vi "2636 EPSC fully synced version.vi"() -> ()   [LabVIEW 2023]
uses:
  <instrlib>/Keithley 2600 Series/Public/Channel.ctl
  <instrlib>/Keithley 2600 Series/Keithley 2600 Series.lvlib
  <userlib>/_OpenG.lib/time/time.llb/openg_time.lvlib
panel:
  in  "error in (no error)":errorcluster
  in  "Log Time After Pulses (s)":dbl=0.5 format="%#_13g"
  in  "Log Time Before Pulses (s)":dbl=0.5 format="%#_13g"
  in  "Auto Enable Output":bool=TRUE
  in  "Reset":bool=TRUE
  in  "Error Query":bool
  out "Pulsed IV Filename Out":path caption="Filename Out"
  in  "Pulsed IV Filename":path=path "C:/Data/pulse_I_V.lvm" caption="Filename"
  out "Pulse IV":cluster{"X":dbl[], "Y":dbl[]}[](graph)
  out "I_ds Log Filename Out":path caption="Filename Out"
  in  "I_ds Log Filename":path=path "C:/Data/I_ds_vs_time.lvm" caption="Filename"
  out "Data":dbl[](array[numeric])
  out "Result Chart":dynamicdata(graph)
  out "error out":errorcluster
  out "Complete?":bool
  out "Overflow?":bool
  in  "Stop":bool
  in  "Pulse Duration (s)":dbl=0.01
  in  "Post-Pulse Duration (s)":dbl=0.05
  in  "Pre-Pulse Duration (s)":dbl=0.05
  in  "Buffer size":u32=1024
  in  "Pulse Number":u32=10
  in  "Drain Source Channel":T1=enum."Channel B"
  in  "V_ds(V)":dbl=0.01
  in  "I_ds NPLC":dbl=0.1
  in  "I_ds Range (A)":dbl=1e-06
  in  "I pulse Range (A)":dbl=1e-06
  in  "I pulse NPLC":dbl=0.1
  in  "Pulse Level (V)":dbl=15.0
  in  "Pulse Channel":T1
  in  "2636 Address":refnum<visa-resource-name>="GPIB0::26::INSTR"
  # "Synaptic EPSC Measurement (Three-terminal Devices)"
  # "by JHC (20250322)"
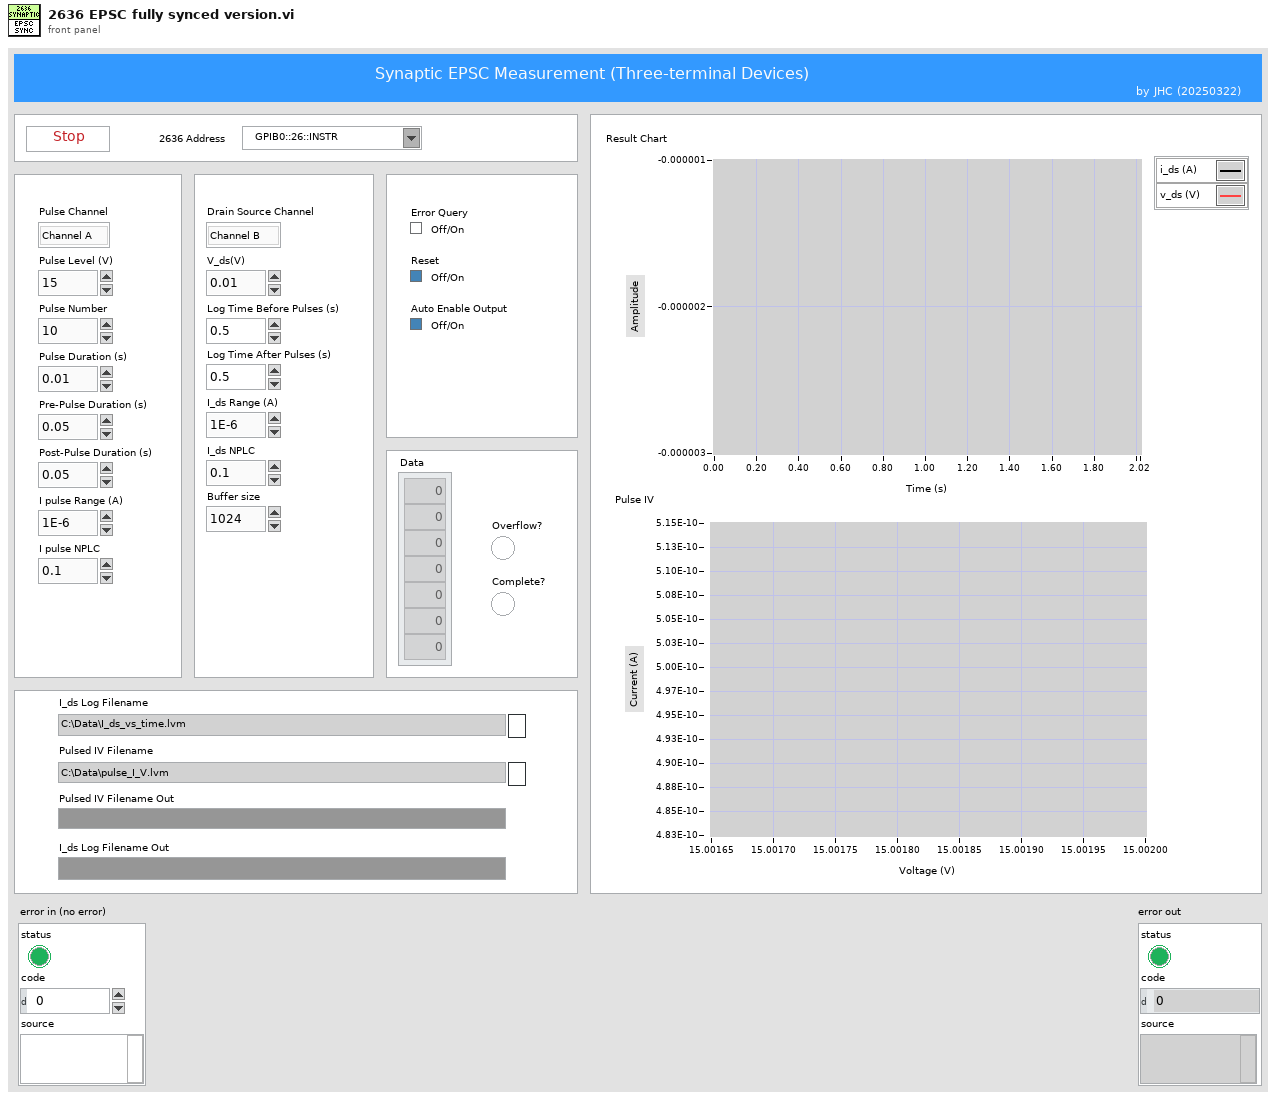
[diagram p1: front panel]
types:
  T1 = typedef "Keithley 2600 Series.lvlib/Channel.ctl" = enum32{"Channel A", "Channel B"}
  T2 = enum16{"None/Disconnect", "Digital I/O Trigger", "TSP-Link Trigger", "LAN Trigger", "Blender", "Timer Expired", "Front Panel Trigger", "Software Trigger", "SMU Sweeping", "SMU Armed", "SMU Source Complete", "SMU Measure Complete", "SMU Pulse Complete", "SMU Sweep Complete", "SMU Idle"}
  T3 = enum16{"Current", "Voltage", "IV", "Resistance", "Power"}
  T4 = enum32{"ASCII", "Real 32", "Real 64", "Single Precision Real", "Double Precision Real"}
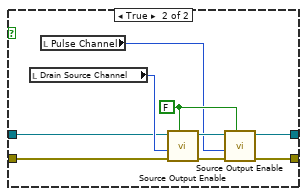
[diagram p2: hidden frame]
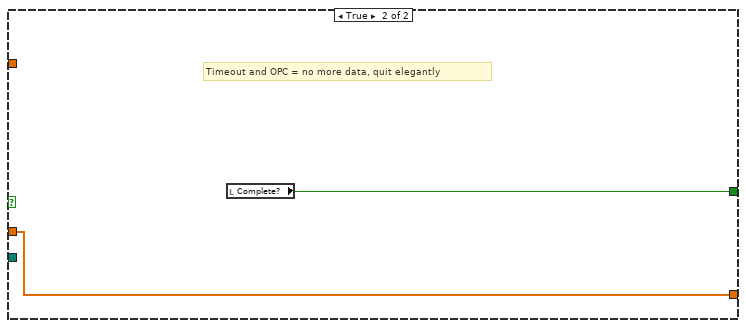
[diagram p5: hidden frame]
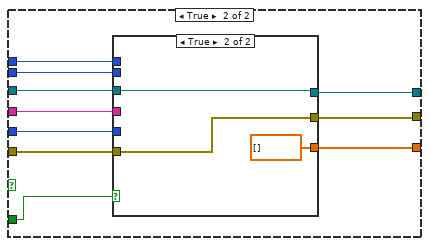
[diagram p8: hidden frame]
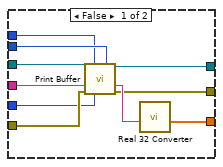
[diagram p9: hidden frame]
diagram:
  w19 = sgl[] [] ("Data Array Out")
  w22 = u16 1 items=["Channel A", "Channel B"] ("Channel (Channel A)")
  w23 = u16 0 items=["Channel A", "Channel B"] ("Channel (Channel A)")
  w39 = u16 0 items=["Current", "Voltage", "Resistance", "Power"] ("Function (Current)")
  w47 = u16 2 items=["Channel A", "Channel B", "Channels A & B", "User"] ("Screen (Channels A & B)")
  # "Wait 1s"
  # "Start Pulse SMU"
  # "Start DS SMU"
  n1 = call <instrlib>:"Initialize.vi"("Reset (True)"="Reset", "error in (no error)"="error in (no error)", "Error Query (False)"="Error Query", "ID Query (True)"=TRUE, "VISA resource name"="2636 Address") -> ("error out"=w2:errorcluster, "VISA resource name out"=w5:refnum<visa-resource-name>)  [unwired: 5 in]
  n2 = call <instrlib>:"Error Queue Clear.vi"("error in (no error)"=w2, "VISA resource name"=w5) -> ("error out"=w3:errorcluster, "VISA resource name out"=w4:refnum<visa-resource-name>)  [unwired: 6 in, 2 out]
  n3 = call <instrlib>:"Abort SMU Op.vi"("error in"=w3, "Channel (Channel A)"=w23, "VISA resource name"=w4) -> ("error out"=w24:errorcluster, "VISA resource name out"=w25:refnum<visa-resource-name>)  [unwired: 5 in, 2 out]
  n4 = call <instrlib>:"Abort SMU Op.vi"("error in"=w24, "Channel (Channel A)"=w22, "VISA resource name"=w25) -> ("error out"=w20:errorcluster, "VISA resource name out"=w21:refnum<visa-resource-name>)  [unwired: 5 in, 2 out]
  n5 = call <instrlib>:"Reset SMU.vi"("SMU B (No)"="Reset", "SMU A (No)"="Reset", "error in (no error)"=w20, "VISA resource name"=w21) -> ("error out"=w86:errorcluster, "VISA resource name out"=w87:refnum<visa-resource-name>)  [unwired: 4 in, 2 out]
  n6 = flat-sequence {
    tunnel: w87 -> [w120]
    tunnel: w86 -> [w119]
    tunnel: [w101] -> w85
    tunnel: [w100] -> w84
    tunnel: w85 -> [w143]
    tunnel: w84 -> [w144]
    tunnel: [w142] -> w83
    tunnel: [w141] -> w82
    tunnel: w83 -> [w184]
    tunnel: w82 -> [w182]
    tunnel: [w163] -> w81
    tunnel: [w162] -> w80
    tunnel: w81 -> [w262]
    tunnel: w80 -> [w261]
    tunnel: [w229] -> w79
    tunnel: [w228] -> w78
    tunnel: [w214] -> w77
    tunnel: w79 -> [w295]
    tunnel: w78 -> [w296]
    tunnel: w77 -> [w318]
    tunnel: [w299] -> w76
    tunnel: [w298] -> w75
    tunnel: w76 -> [w326]
    tunnel: w75 -> [w325]
    tunnel: [w322] -> w44
    tunnel: [w321] -> w43
    frame #0 {
      w108 = enum32{"Current", "Voltage"}."Current" ("Function (Current)")
      w109 = FALSE ("Autorange (On)")
      w89 = enum32{"Current", "Voltage"}."Voltage" ("Function (Current)")
      # "Init Pulse Gate Channel"
      n7 = call <instrlib>:"Source Function.vi"("Function (Current)"=w89, "error in (no error)"=w119, "Channel (Channel A)"="Pulse Channel", "VISA resource name"=w120) -> ("error out"=w121:errorcluster, "VISA resource name out"=w122:refnum<visa-resource-name>)  [unwired: 4 in, 2 out]
      n8 = call <instrlib>:"Source Level.vi"("Level (0.000)"=0.0, "Function (Current)"=w89, "error in (no error)"=w121, "Channel (Channel A)"="Pulse Channel", "VISA resource name"=w122) -> ("error out"=w117:errorcluster, "VISA resource name out"=w118:refnum<visa-resource-name>)  [unwired: 3 in, 2 out]
      n9 = call <instrlib>:"Source Autorange.vi"("Autorange (On)"=w109, "Function (Current)"=w89, "error in (no error)"=w117, "Channel (Channel A)"="Pulse Channel", "VISA resource name"=w118) -> ("error out"=w115:errorcluster, "VISA resource name out"=w116:refnum<visa-resource-name>)  [unwired: 3 in, 2 out]
      n10 = local read "Pulse Level (V)"() -> (w88:dbl)
      n11 = call <instrlib>:"Source Autorange.vi"("Autorange (On)"=w109, "Function (Current)"=w108, "error in (no error)"=w115, "Channel (Channel A)"="Pulse Channel", "VISA resource name"=w116) -> ("error out"=w96:errorcluster, "VISA resource name out"=w98:refnum<visa-resource-name>)  [unwired: 3 in, 2 out]
      n12 = call <instrlib>:"Source Range.vi"("Range (1.000)"=w88, "Function (Current)"=w89, "error in (no error)"=w96, "Channel (Channel A)"="Pulse Channel", "VISA resource name"=w98) -> ("error out"=w95:errorcluster, "VISA resource name out"=w97:refnum<visa-resource-name>)  [unwired: 3 in, 2 out]
      n13 = call <instrlib>:"Measure NPLC.vi"("NPLC (1.000)"="I pulse NPLC", "error in (no error)"=w95, "Channel (Channel A)"="Pulse Channel", "VISA resource name"=w97) -> ("error out"=w113:errorcluster, "VISA resource name out"=w110:refnum<visa-resource-name>)  [unwired: 4 in, 2 out]
      n14 = call <instrlib>:"Measure Autorange.vi"("Autorange (On)"=w109, "Function (Current)"=w89, "error in (no error)"=w113, "Channel (Channel A)"="Pulse Channel", "VISA resource name"=w110) -> ("error out"=w112:errorcluster, "VISA resource name out"=w111:refnum<visa-resource-name>)  [unwired: 3 in, 2 out]
      n15 = call <instrlib>:"Measure Autorange.vi"("Autorange (On)"=w109, "Function (Current)"=w108, "error in (no error)"=w112, "Channel (Channel A)"="Pulse Channel", "VISA resource name"=w111) -> ("error out"=w94:errorcluster, "VISA resource name out"=w93:refnum<visa-resource-name>)  [unwired: 3 in, 2 out]
      n16 = call <instrlib>:"Measure Range.vi"("Range (1.000)"=w88, "Function (Current)"=w89, "error in (no error)"=w94, "Channel (Channel A)"="Pulse Channel", "VISA resource name"=w93) -> ("error out"=w91:errorcluster, "VISA resource name out"=w92:refnum<visa-resource-name>)  [unwired: 3 in, 2 out]
      n17 = call <instrlib>:"Measure Range.vi"("Range (1.000)"="I pulse Range (A)", "Function (Current)"=w108, "error in (no error)"=w91, "Channel (Channel A)"="Pulse Channel", "VISA resource name"=w92) -> ("error out"=w106:errorcluster, "VISA resource name out"=w105:refnum<visa-resource-name>)  [unwired: 3 in, 2 out]
      n18 = call <instrlib>:"Measure Sense Mode.vi"("error in (no error)"=w106, "Channel (Channel A)"="Pulse Channel", "VISA resource name"=w105) -> ("error out"=w103:errorcluster, "VISA resource name out"=w104:refnum<visa-resource-name>)  [unwired: 2 in, 5 out]
      n19 = call <instrlib>:"Measure Autozero.vi"("Autozero (Auto)"=enum32{"Off", "Once", "Auto"}."Once", "error in (no error)"=w103, "Channel (Channel A)"="Pulse Channel", "VISA resource name"=w104) -> ("error out"=w100:errorcluster, "VISA resource name out"=w101:refnum<visa-resource-name>)  [unwired: 1 in, 5 out]
    }
    frame #1 {
      w126 = 0.0 ("Interval (0.000)")
      w146 = enum32{"Current", "Voltage"}."Current" ("Function (Current)")
      w145 = FALSE ("Autorange (On)")
      w132 = enum32{"Current", "Voltage"}."Voltage" ("Function (Current)")
      # "Init Drain Source Channel"
      n20 = call <instrlib>:"Source Function.vi"("Function (Current)"=w132, "error in (no error)"=w144, "Channel (Channel A)"="Drain Source Channel", "VISA resource name"=w143) -> ("error out"=w160:errorcluster, "VISA resource name out"=w161:refnum<visa-resource-name>)  [unwired: 4 in, 2 out]
      n21 = call <instrlib>:"Source Level.vi"("Level (0.000)"="V_ds(V)", "Function (Current)"=w132, "error in (no error)"=w160, "Channel (Channel A)"="Drain Source Channel", "VISA resource name"=w161) -> ("error out"=w158:errorcluster, "VISA resource name out"=w159:refnum<visa-resource-name>)  [unwired: 3 in, 2 out]
      n22 = call <instrlib>:"Source Autorange.vi"("Autorange (On)"=w145, "Function (Current)"=w132, "error in (no error)"=w158, "Channel (Channel A)"="Drain Source Channel", "VISA resource name"=w159) -> ("error out"=w156:errorcluster, "VISA resource name out"=w157:refnum<visa-resource-name>)  [unwired: 3 in, 2 out]
      n23 = call <instrlib>:"Source Autorange.vi"("Autorange (On)"=w145, "Function (Current)"=w146, "error in (no error)"=w156, "Channel (Channel A)"="Drain Source Channel", "VISA resource name"=w157) -> ("error out"=w140:errorcluster, "VISA resource name out"=w137:refnum<visa-resource-name>)  [unwired: 3 in, 2 out]
      n24 = call <instrlib>:"Source Range.vi"("Range (1.000)"="V_ds(V)", "Function (Current)"=w132, "error in (no error)"=w140, "Channel (Channel A)"="Drain Source Channel", "VISA resource name"=w137) -> ("error out"=w139:errorcluster, "VISA resource name out"=w138:refnum<visa-resource-name>)  [unwired: 3 in, 2 out]
      n25 = call <instrlib>:"Measure NPLC.vi"("NPLC (1.000)"="I_ds NPLC", "error in (no error)"=w139, "Channel (Channel A)"="Drain Source Channel", "VISA resource name"=w138) -> ("error out"=w127:errorcluster, "VISA resource name out"=w128:refnum<visa-resource-name>)  [unwired: 4 in, 2 out]
      n26 = call <instrlib>:"Measure Interval.vi"("Interval (0.000)"=w126, "error in (no error)"=w127, "Channel (Channel A)"="Drain Source Channel", "VISA resource name"=w128) -> ("error out"=w130:errorcluster, "VISA resource name out"=w129:refnum<visa-resource-name>)  [unwired: 4 in, 2 out]
      n27 = call <instrlib>:"Measure Delay.vi"("Delay (0)"=w126, "error in (no error)"=w130, "Channel (Channel A)"="Drain Source Channel", "VISA resource name"=w129) -> ("error out"=w124:errorcluster, "VISA resource name out"=w125:refnum<visa-resource-name>)  [unwired: 4 in, 2 out]
      n28 = call <instrlib>:"Measure Autorange.vi"("Autorange (On)"=w145, "Function (Current)"=w132, "error in (no error)"=w124, "Channel (Channel A)"="Drain Source Channel", "VISA resource name"=w125) -> ("error out"=w154:errorcluster, "VISA resource name out"=w153:refnum<visa-resource-name>)  [unwired: 3 in, 2 out]
      n29 = call <instrlib>:"Measure Autorange.vi"("Autorange (On)"=w145, "Function (Current)"=w146, "error in (no error)"=w154, "Channel (Channel A)"="Drain Source Channel", "VISA resource name"=w153) -> ("error out"=w133:errorcluster, "VISA resource name out"=w134:refnum<visa-resource-name>)  [unwired: 3 in, 2 out]
      n30 = call <instrlib>:"Measure Range.vi"("Range (1.000)"="V_ds(V)", "Function (Current)"=w132, "error in (no error)"=w133, "Channel (Channel A)"="Drain Source Channel", "VISA resource name"=w134) -> ("error out"=w136:errorcluster, "VISA resource name out"=w135:refnum<visa-resource-name>)  [unwired: 3 in, 2 out]
      n31 = call <instrlib>:"Measure Range.vi"("Range (1.000)"="I_ds Range (A)", "Function (Current)"=w146, "error in (no error)"=w136, "VISA resource name"=w135) -> ("error out"=w151:errorcluster, "VISA resource name out"=w150:refnum<visa-resource-name>)  [unwired: 4 in, 2 out]
      n32 = call <instrlib>:"Measure Sense Mode.vi"("error in (no error)"=w151, "Channel (Channel A)"="Drain Source Channel", "VISA resource name"=w150) -> ("error out"=w148:errorcluster, "VISA resource name out"=w149:refnum<visa-resource-name>)  [unwired: 2 in, 5 out]
      n33 = call <instrlib>:"Measure Autozero.vi"("Autozero (Auto)"=enum32{"Off", "Once", "Auto"}."Once", "error in (no error)"=w148, "Channel (Channel A)"="Drain Source Channel", "VISA resource name"=w149) -> ("error out"=w142:errorcluster, "VISA resource name out"=w141:refnum<visa-resource-name>)  [unwired: 1 in, 5 out]
    }
    frame #2 {
      w176 = TRUE ("Append Mode (Off)")
      w175 = "v_ds" ("Buffer Name (buf)")
      w177 = TRUE ("Append Mode (Off)")
      w179 = "i_ds" ("Buffer Name (buf)")
      w188 = FALSE ("Collect Timestamps (Off)")
      w187 = "pulse_iv_table.v" ("Buffer Name (buf)")
      w186 = TRUE ("Append Mode (Off)")
      w185 = "pulse_iv_table.i" ("Buffer Name (buf)")
      # "set up circular buffer"
      # "A large size"
      # "Init Buffer"
      n34 = local read "Pulse Channel"() -> (w203:T1)
      n35 = VISA Write(VISA resource name=w182, write buffer="pulse_iv_table = {}\nds_iv_table = {}", error in (no error)=w184) -> (VISA resource name out=w189:refnum<visa-resource-name>, error out=w190:errorcluster)  [unwired: 1 out]
      n36 = call <instrlib>:"Error Query.vi"("error in (no error)"=w190, "VISA resource name"=w189) -> ("error out"=w202:errorcluster, "VISA resource name out"=w201:refnum<visa-resource-name>)  [unwired: 8 out]
      n37 = call <instrlib>:"Buffer Make Buffer.vi"("Capacity (1)"="Pulse Number", "Channel (Channel A)"=w203, "error in (no error)"=w202, "Buffer Name (buf)"=w185, "VISA resource name"=w201) -> ("error out"=w191:errorcluster, "VISA resource name out"=w192:refnum<visa-resource-name>)  [unwired: 1 in, 4 out]
      n38 = call <instrlib>:"Buffer Clear.vi"("error in (no error)"=w191, "Buffer Name"=w185, "VISA resource name"=w192) -> ("error out"=w194:errorcluster, "VISA resource name out"=w193:refnum<visa-resource-name>)  [unwired: 7 out]
      n39 = call <instrlib>:"Buffer Configure.vi"("Collect Timestamps (Off)"=w188, "error in (no error)"=w194, "Buffer Name"=w185, "Append Mode (Off)"=w186, "VISA resource name"=w193) -> ("error out"=w196:errorcluster, "VISA resource name out"=w195:refnum<visa-resource-name>)  [unwired: 2 in, 3 out]
      n40 = call <instrlib>:"Buffer Make Buffer.vi"("Capacity (1)"="Pulse Number", "Channel (Channel A)"=w203, "error in (no error)"=w196, "Buffer Name (buf)"=w187, "VISA resource name"=w195) -> ("error out"=w198:errorcluster, "VISA resource name out"=w197:refnum<visa-resource-name>)  [unwired: 1 in, 4 out]
      n41 = call <instrlib>:"Buffer Clear.vi"("error in (no error)"=w198, "Buffer Name"=w187, "VISA resource name"=w197) -> ("error out"=w200:errorcluster, "VISA resource name out"=w199:refnum<visa-resource-name>)  [unwired: 7 out]
      n42 = call <instrlib>:"Buffer Configure.vi"("Collect Source Values (Off)"=w188, "error in (no error)"=w200, "Buffer Name"=w187, "Append Mode (Off)"=w186, "VISA resource name"=w199) -> ("error out"=w210:errorcluster, "VISA resource name out"=w209:refnum<visa-resource-name>)  [unwired: 2 in, 3 out]
      n43 = local read "Drain Source Channel"() -> (w167:T1)
      n44 = call <instrlib>:"Buffer Make Buffer.vi"("Capacity (1)"="Buffer size", "Channel (Channel A)"=w167, "error in (no error)"=w210, "Buffer Name (buf)"=w179, "VISA resource name"=w209) -> ("error out"=w206:errorcluster, "VISA resource name out"=w205:refnum<visa-resource-name>)  [unwired: 1 in, 4 out]
      n45 = call <instrlib>:"Buffer Clear.vi"("error in (no error)"=w206, "Buffer Name"=w179, "VISA resource name"=w205) -> ("error out"=w208:errorcluster, "VISA resource name out"=w207:refnum<visa-resource-name>)  [unwired: 7 out]
      n46 = call <instrlib>:"Buffer Configure.vi"("Collect Timestamps (Off)"=w177, "error in (no error)"=w208, "Buffer Name"=w179, "Append Mode (Off)"=w177, "VISA resource name"=w207) -> ("error out"=w181:errorcluster, "VISA resource name out"=w180:refnum<visa-resource-name>)  [unwired: 2 in, 3 out]
      n47 = call <instrlib>:"Advanced Buffer Configuration.vi"("VISA resource name"=w180, "Enable Buffer Cache Mode (Disable)"=w177, "Buffer Name"=w179, "Buffer Fill Mode (Fill_Once)"=enum16{"FILL_ONCE", "FILL_WINDOW"}."FILL_WINDOW", "error in (no error)"=w181) -> ("VISA resource name out"=w165:refnum<visa-resource-name>, "error out"=w164:errorcluster)  [unwired: 9 in]
      n48 = call <instrlib>:"Buffer Make Buffer.vi"("Capacity (1)"="Buffer size", "Channel (Channel A)"=w167, "error in (no error)"=w164, "Buffer Name (buf)"=w175, "VISA resource name"=w165) -> ("error out"=w171:errorcluster, "VISA resource name out"=w172:refnum<visa-resource-name>)  [unwired: 1 in, 4 out]
      n49 = call <instrlib>:"Buffer Clear.vi"("error in (no error)"=w171, "Buffer Name"=w175, "VISA resource name"=w172) -> ("error out"=w169:errorcluster, "VISA resource name out"=w170:refnum<visa-resource-name>)  [unwired: 7 out]
      n50 = call <instrlib>:"Buffer Configure.vi"("Collect Timestamps (Off)"=w176, "error in (no error)"=w169, "Buffer Name"=w175, "Append Mode (Off)"=w176, "VISA resource name"=w170) -> ("error out"=w173:errorcluster, "VISA resource name out"=w174:refnum<visa-resource-name>)  [unwired: 2 in, 3 out]
      n51 = call <instrlib>:"Advanced Buffer Configuration.vi"("VISA resource name"=w174, "Enable Buffer Cache Mode (Disable)"=w176, "Buffer Name"=w175, "Buffer Fill Mode (Fill_Once)"=enum16{"FILL_ONCE", "FILL_WINDOW"}."FILL_WINDOW", "error in (no error)"=w173) -> ("VISA resource name out"=w162:refnum<visa-resource-name>, "error out"=w163:errorcluster)  [unwired: 9 in]
    }
    frame #3 {
      w218 = u32 4 ("Timer Number (1)")
      w232 = u32 1 ("Timer Number (1)")
      w244 = u32 3 ("Timer Number (1)")
      w268 = u32 2 ("Timer Number (1)")
      # "SMU Armed when timer4 expires"
      # "Trigger timer4 when the SMU Sweeping, only once"
      # "Trigger timer1 when the SMU Armed, repeat N times"
      # "Trigger end pulse after timer3 expired"
      # "Configure measure action (default is 0) to start after source immediately"
      # "set source pulse level and end pusle idle"
      # "Trigger timer3 when the SMU source pulse level"
      # "Create a fixed level voltage sweep"
      # "Configure source action to start after timer2 expired"
      # "Trigger timer2 when timer1 expired or first run."
      # "Init Trigger Model (Pulse Channel)"
      n52 = local read "Pulse Channel"() -> (w214:T1)
      n53 = Pick Line(multi-line string="smua\nsmub", line index=w214) -> (output string=w227:string)  [unwired: 1 in]
      n54 = Format Into String(format string="%s.trigger.source.listv({%f})\\n", w227, "Pulse Level (V)") -> (resulting string=w265:string)  [unwired: 2 in, 1 out]
      n55 = call <instrlib>:"Format Event ID.vi"("Channel (Channel A)"=w214, "Event Type (None)"=T2."SMU Sweeping") -> ("Event ID"=w222:string)  [unwired: 8 in, 1 out]
      n56 = Format Into String(format string="%s.trigger.source.action = %s.ENABLE\n%s.trigger.endpulse.action = %s.SOURCE_IDLE", initial string=w265, w227, w227, w227, w227) -> (resulting string=w260:string)  [unwired: 1 in, 1 out]
      n57 = VISA Write(VISA resource name=w261, write buffer=w260, error in (no error)=w262) -> (VISA resource name out=w224:refnum<visa-resource-name>, error out=w223:errorcluster)  [unwired: 1 out]
      n58 = call <instrlib>:"Config Timer.vi"("VISA resource name"=w224, "Delay (1e-3)"="Log Time Before Pulses (s)", "Timer Number (1)"=w218, "error in"=w223, "Input Event"=w222) -> ("VISA resource name out"=w220:refnum<visa-resource-name>, "error out"=w216:errorcluster)  [unwired: 7 in, 2 out]
      n59 = call <instrlib>:"Format Event ID.vi"("Event Module # (1)"=w218, "Event Type (None)"=T2."Timer Expired") -> ("Event ID"=w217:string)  [unwired: 8 in, 1 out]
      n60 = call <instrlib>:"Config Arm Event.vi"("Arm Input Event"=w217, "error in"=w216, "Channel (Channel A)"=w214, "VISA resource name"=w220) -> ("error out"=w212:errorcluster, "VISA resource name out"=w211:refnum<visa-resource-name>)  [unwired: 4 in, 2 out]
      n61 = call <instrlib>:"Format Event ID.vi"("Channel (Channel A)"=w214, "Event Type (None)"=T2."SMU Armed") -> ("Event ID"=w213:string)  [unwired: 8 in, 1 out]
      n62 = local read "Pre-Pulse Duration (s)"() -> (w241:dbl)
      n63 = local read "Pulse Number"() -> (w237:u32)
      n64 = local read "Pulse Duration (s)"() -> (w242:dbl)
      n65 = Decrement(x=w237) -> (x-1=w233:u32)
      n66 = Compound Arithmetic op=ADD(w242, w241, "Post-Pulse Duration (s)") -> (w239:dbl)
      n67 = call <instrlib>:"Config Timer.vi"("VISA resource name"=w211, "Count (1)"=w233, "Delay (1e-3)"=w239, "Timer Number (1)"=w232, "Passthrough (Off)"=TRUE, "error in"=w212, "Input Event"=w213) -> ("VISA resource name out"=w234:refnum<visa-resource-name>, "error out"=w235:errorcluster)  [unwired: 5 in, 2 out]
      n68 = call <instrlib>:"Format Event ID.vi"("Event Module # (1)"=w232, "Event Type (None)"=T2."Timer Expired") -> ("Event ID"=w272:string)  [unwired: 8 in, 1 out]
      n69 = call <instrlib>:"Config Timer.vi"("VISA resource name"=w234, "Delay (1e-3)"="Pre-Pulse Duration (s)", "Timer Number (1)"=w268, "error in"=w235, "Input Event"=w272) -> ("VISA resource name out"=w271:refnum<visa-resource-name>, "error out"=w270:errorcluster)  [unwired: 7 in, 2 out]
      n70 = call <instrlib>:"Format Event ID.vi"("Event Module # (1)"=w268, "Event Type (None)"=T2."Timer Expired") -> ("Event ID"=w267:string)  [unwired: 8 in, 1 out]
      n71 = call <instrlib>:"Config Source Event.vi"("Input Event"=w267, "error in"=w270, "Channel (Channel A)"=w214, "VISA resource name"=w271) -> ("error out"=w255:errorcluster, "VISA resource name out"=w256:refnum<visa-resource-name>)  [unwired: 4 in, 2 out]
      n72 = call <instrlib>:"Format Event ID.vi"("Channel (Channel A)"=w214, "Event Type (None)"=T2."SMU Source Complete") -> ("Event ID"=w258:string)  [unwired: 8 in, 1 out]
      n73 = call <instrlib>:"Config Timer.vi"("VISA resource name"=w256, "Delay (1e-3)"="Pulse Duration (s)", "Timer Number (1)"=w244, "error in"=w255, "Input Event"=w258) -> ("VISA resource name out"=w254:refnum<visa-resource-name>, "error out"=w253:errorcluster)  [unwired: 7 in, 2 out]
      n74 = call <instrlib>:"Config Measure Event.vi"("VISA resource name"=w254, "Configure Measurement (Disable)"=enum8{"DISABLE", "ENABLE", "ASYNC"}."ENABLE", "Buffer 1"="pulse_iv_table.i" ("Buffer Name (buf)"), "Buffer 2"="pulse_iv_table.v" ("Buffer Name (buf)"), "Channel (Channel A)"=w214, "Function (Current)"=T3."IV", "error in"=w253, "Measure Input Event"="0") -> ("VISA resource name out"=w247:refnum<visa-resource-name>, "error out"=w246:errorcluster)  [unwired: 4 in, 2 out]
      n75 = call <instrlib>:"Format Event ID.vi"("Event Module # (1)"=w244, "Event Type (None)"=T2."Timer Expired") -> ("Event ID"=w243:string)  [unwired: 8 in, 1 out]
      n76 = local read "Pulse Number"() -> (w225:u32)
      n77 = call <instrlib>:"Config End Pulse Event.vi"("Input Event"=w243, "error in"=w246, "Channel (Channel A)"=w214, "VISA resource name"=w247) -> ("error out"=w231:errorcluster, "VISA resource name out"=w230:refnum<visa-resource-name>)  [unwired: 4 in, 2 out]
      n78 = call <instrlib>:"Config Layer Count.vi"("Trigger Count (1)"=w225, "Arm Count (1)"=u32 1 ("Trigger Count (1)"), "error in"=w231, "Channel (Channel A)"=w214, "VISA resource name"=w230) -> ("error out"=w228:errorcluster, "VISA resource name out"=w229:refnum<visa-resource-name>)  [unwired: 3 in, 2 out]
    }
    frame #4 {
      w280 = u32 5 ("Timer Number (1)")
      w308 = u32 1 ("Blender Number (1)")
      # "BUG from Driver: if Async, measure.Y is not set"
      # "No trigger, start\nasync measure after SMU Armed, as fast as possible"
      # "Trigger timer5 when Pulse SMU Idle\nto keep measure for a while"
      # "Blend two events from Pulse SMU to trigger DS SMU Source action\nDS SMU Source start when Pulse SMU start sweeping\nWhen Pulse SMU become idle, DS SMU source again and stop"
      # "set source level, and hold"
      # "Create a fixed level voltage sweep"
      # "Init Trigger Model (Drain Source Channel)"
      n79 = local read "Drain Source Channel"() -> (w301:T1)
      n80 = local read "V_ds(V)"() -> (w312:dbl)
      n81 = Pick Line(multi-line string="smua\nsmub", line index=w301) -> (output string=w288:string)  [unwired: 1 in]
      n82 = Format Into String(format string="%s.trigger.source.listv({%f})\\n", w288, w312) -> (resulting string=w315:string)  [unwired: 2 in, 1 out]
      n83 = Format Into String(format string="%s.trigger.source.action = %s.ENABLE\n%s.trigger.endpulse.action = %s.SOURCE_HOLD", initial string=w315, w288, w288, w288, w288) -> (resulting string=w294:string)  [unwired: 1 in, 1 out]
      n84 = VISA Write(VISA resource name=w295, write buffer=w294, error in (no error)=w296) -> (VISA resource name out=w284:refnum<visa-resource-name>, error out=w285:errorcluster)  [unwired: 1 out]
      n85 = call <instrlib>:"Format Event ID.vi"("Channel (Channel A)"=w318, "Event Type (None)"=T2."SMU Sweeping") -> ("Event ID"=w279:string)  [unwired: 8 in, 1 out]
      n86 = call <instrlib>:"Format Event ID.vi"("Channel (Channel A)"=w318, "Event Type (None)"=T2."SMU Idle") -> ("Event ID"=w282:string)  [unwired: 8 in, 1 out]
      n87 = call <instrlib>:"Config Timer.vi"("VISA resource name"=w284, "Delay (1e-3)"="Log Time After Pulses (s)", "Timer Number (1)"=w280, "error in"=w285, "Input Event"=w282) -> ("VISA resource name out"=w276:refnum<visa-resource-name>, "error out"=w277:errorcluster)  [unwired: 7 in, 2 out]
      n88 = call <instrlib>:"Format Event ID.vi"("Event Module # (1)"=w280, "Event Type (None)"=T2."Timer Expired") -> ("Event ID"=w278:string)  [unwired: 8 in, 1 out]
      n89 = call <instrlib>:"Config Event Blender.vi"("VISA resource name"=w276, "Input Event 1"=w278, "Input Event 2"=w279, "Blender Number (1)"=w308, "Blend Type (OR)"=enum16{"OR", "AND"}."OR", "error in"=w277) -> ("VISA resource name out"=w310:refnum<visa-resource-name>, "error out"=w311:errorcluster)  [unwired: 6 in, 2 out]
      n90 = call <instrlib>:"Format Event ID.vi"("Event Module # (1)"=w308, "Event Type (None)"=T2."Blender") -> ("Event ID"=w307:string)  [unwired: 8 in, 1 out]
      n91 = call <instrlib>:"Config Source Event.vi"("Input Event"=w307, "error in"=w311, "Channel (Channel A)"=w301, "VISA resource name"=w310) -> ("error out"=w304:errorcluster, "VISA resource name out"=w305:refnum<visa-resource-name>)  [unwired: 4 in, 2 out]
      n92 = call <instrlib>:"Config Measure Event.vi"("VISA resource name"=w305, "Configure Measurement (Disable)"=enum8{"DISABLE", "ENABLE", "ASYNC"}."ENABLE", "Buffer 1"="i_ds" ("Buffer Name (buf)"), "Buffer 2"="v_ds" ("Buffer Name (buf)"), "Channel (Channel A)"=w301, "Function (Current)"=T3."IV", "error in"=w304) -> ("VISA resource name out"=w290:refnum<visa-resource-name>, "error out"=w291:errorcluster)  [unwired: 5 in, 2 out]
      n93 = Format Into String(format string="%s.trigger.measure.action = %s.ASYNC", w288, w288) -> (resulting string=w287:string)  [unwired: 2 in, 1 out]
      n94 = VISA Write(VISA resource name=w290, write buffer=w287, error in (no error)=w291) -> (VISA resource name out=w293:refnum<visa-resource-name>, error out=w292:errorcluster)  [unwired: 1 out]
      n95 = call <instrlib>:"Config Layer Count.vi"("Trigger Count (1)"=u32 2 ("Arm Count (1)"), "Arm Count (1)"=u32 1, "error in"=w292, "Channel (Channel A)"=w301, "VISA resource name"=w293) -> ("error out"=w298:errorcluster, "VISA resource name out"=w299:refnum<visa-resource-name>)  [unwired: 3 in, 2 out]
    }
    frame #5 {
      # "Other init jobs"
      n96 = call <instrlib>:"Data Output Format.vi"("ASCII Precision (6)"=6, "error in (no error)"=w325, "Data Format (ASCII)"=T4."Real 32", "VISA resource name"=w326) -> ("error out"=w321:errorcluster, "VISA resource name out"=w322:refnum<visa-resource-name>)  [unwired: 4 in, 2 out]
    }
  }
  n97 = local read "Pulse Channel"() -> (w41:T1)
  n98 = local read "Drain Source Channel"() -> (w40:T1)
  n99 = call <instrlib>:"Display Screen.vi"("Screen (Channels A & B)"=w47, "error in (no error)"=w43, "VISA resource name"=w44) -> ("error out"=w50:errorcluster, "Node Out"=w49:string, "VISA resource name out"=w48:refnum<visa-resource-name>)  [unwired: 5 in, 1 out]
  n100 = call <instrlib>:"Display Measure Function.vi"("Function (Current)"=w39, "error in (no error)"=w50, "Channel (Channel A)"=w41, "Node In"=w49, "VISA resource name"=w48) -> ("error out"=w46:errorcluster, "VISA resource name out"=w45:refnum<visa-resource-name>)  [unwired: 3 in, 2 out]
  n101 = control-ref of="Overflow?"() -> (w36:refnum<vi>)
  n102 = control-ref of="Complete?"() -> (w35:refnum<vi>)
  n103 = control-ref of="Stop"() -> (w30:refnum<vi>)
  n104 = call <instrlib>:"Display Measure Function.vi"("Function (Current)"=w39, "error in (no error)"=w46, "Channel (Channel A)"=w40, "VISA resource name"=w45) -> ("error out"=w42:errorcluster, "VISA resource name out"=w38:refnum<visa-resource-name>)  [unwired: 4 in, 2 out]
  n105 = Build Array(w36, w35, w30) -> (w34:refnum<vi>[])
  n106 = case shown="True" "Auto Enable Output" {
    tunnel: [w327 w337] -> w9
    tunnel: [w328 w336] -> w10
    tunnel: w42 -> [w327 w332]
    tunnel: w41 -> [_ w331]
    tunnel: w40 -> [_ w330]
    tunnel: w38 -> [w328 w329]
    frame False {
    }
    frame True {
      w333 = TRUE ("Output (Off)")
      n107 = call <instrlib>:"Source Output Enable.vi"("Output (Off)"=w333, "error in (no error)"=w332, "Channel (Channel A)"=w330, "VISA resource name"=w329) -> ("error out"=w335:errorcluster, "VISA resource name out"=w334:refnum<visa-resource-name>)  [unwired: 4 in, 2 out]
      n108 = call <instrlib>:"Source Output Enable.vi"("Output (Off)"=w333, "error in (no error)"=w335, "Channel (Channel A)"=w331, "VISA resource name"=w334) -> ("error out"=w337:errorcluster, "VISA resource name out"=w336:refnum<visa-resource-name>)  [unwired: 4 in, 2 out]
    }
  }
  n109 = for {
    tunnel: w34 -> [w339] mode=indexing
    tunnel: [w338] -> w31
    # "Init GUI"
    n110 = invoke class="Bool (strict)" method="Reinit To Default"(reference=w339) -> (error out=w338:errorcluster)  [unwired: 2 in, 2 out]
  }
  n111 = call <userlib>:"Wait (ms)__ogtk.vi"("error in (no error)"=w9, "milliseconds to wait"=u32 1000) -> ("error out"=w8:errorcluster)  [unwired: 8 in, 1 out]
  n112 = call <instrlib>:"Initiate Sweep.vi"("error in"=w8, "Channel (Channel A)"=w40, "VISA resource name"=w10) -> ("error out"=w70:errorcluster, "VISA resource name out"=w71:refnum<visa-resource-name>)  [unwired: 5 in, 2 out]
  n113 = Obtain Queue(max queue size (-1, unlimited)=1024, name (unnamed)="data_q", element data type=w19, error in (no error)=w42) -> (queue out=w57:refnum<queue>, error out=w32:errorcluster)  [unwired: 1 in, 1 out]
  n114 = Format Into String(format string="%s, %s, %s", "i_ds" ("Buffer Name(s)"), "i_ds.timestamps" ("Buffer Name(s)"), "v_ds" ("Buffer Name(s)")) -> (resulting string=w74:string)  [unwired: 2 in, 1 out]
  n115 = call <instrlib>:"Initiate Sweep.vi"("error in"=w70, "Channel (Channel A)"=w41, "VISA resource name"=w71) -> ("error out"=w73:errorcluster, "VISA resource name out"=w72:refnum<visa-resource-name>)  [unwired: 5 in, 2 out]
  n116 = Merge Errors(w32, w31) -> (w33:errorcluster)
  n117 = while {
    tunnel: w57 -> [w351]
    tunnel: "I_ds Log Filename" -> [w347]
    tunnel: w33 -> [w350]
    tunnel: [w346] -> w29
    shift-right: [w340] -> w15
    shift-left: w19 -> [w341]
    stop <- w344 stop-if-true
    # "Plot and save I_ds and v_ds"
    n118 = Dequeue Element(queue=w351, timeout in ms (-1)=500, error in (no error)=w350) -> (queue out=w346:refnum<queue>, element=w348:sgl[], timed out?=w349:bool, error out=w343:errorcluster)
    n119 = case shown="False" w349 {
      tunnel: w348 -> [w354 _]
      tunnel: w347 -> [w363 _]
      tunnel: [FALSE ("Operation Complete") w376] -> w342
      tunnel: w341 -> [w355 w375]
      tunnel: [w353 w375] -> w340
      frame False {
        n120 = Decimate 1D Array(w354) -> (w360:sgl[], w359:sgl[], w358:sgl[])
        n121 = for {
          tunnel: [w372] -> w362
          tunnel: [w367] -> w357 mode=indexing
          tunnel: w360 -> [w366] mode=indexing
          tunnel: w359 -> [w365] mode=indexing
          tunnel: w358 -> [w370] mode=indexing
          n122 = To Time Stamp(1:w365) -> (0:w371:timestamp)
          n123 = Build Array(w366) -> (w369:sgl[])
          n124 = Build Array(w370) -> (w368:sgl[])
          n125 = Build Array(w365, w366, w370) -> (w367:sgl[])
          "Data" <- w367
          n126 = Bundle By Name("Y"=w369, "t0"=w371) -> (w374:waveform(sgl))  [unwired: 1 in]
          n127 = Bundle By Name("Y"=w368, "t0"=w371) -> (w373:waveform(sgl))  [unwired: 1 in]
          n128 = Merge Signals(w374, w373) -> (w372:dynamicdata)
        }
        "Result Chart" <- w362
        n129 = Build Array (concatenate)(w355, w354) -> (w353:sgl[])
        n130 = call "Convert to Dynamic Data3"("2D Array"=w357) -> ("Dynamic Data Type"=w361:dynamicdata)  [unwired: 3 in]
        n131 = call "Write To Measurement File"("Signals"=w361, "Filename"=w363) -> ("Filename Out"=→"I_ds Log Filename Out":path)  [unwired: 15 in, 2 out]
      }
      frame True {
        # "Timeout and OPC = no more data, quit elegantly"
        n132 = local read "Complete?"() -> (w376:bool)
      }
    }
    n133 = local read "Stop"() -> (w345:bool)
    n134 = Compound Arithmetic op=OR(w342, w345, w343) -> (w344:bool)
  }
  n135 = while {
    tunnel: w72 -> [w385]
    tunnel: w73 -> [w384]
    shift-right: [w379] -> _
    shift-left: u32 1 ("Start Index (1)") -> [w378]
    tunnel: w74 -> [w401]
    tunnel: "tostring(i_ds.next), tostring(v_ds.next)" ("format string") -> [w399]
    tunnel: w57 -> [w383]
    tunnel: [w398] -> w61
    tunnel: [w382] -> w60
    tunnel: [w386] -> w53
    stop <- w387 stop-if-true
    # "Fetch buffer data and parse dataframes"
    n136 = Wait (ms)(milliseconds to wait=u32 100) -> ()  [unwired: 1 out]
    n137 = VISA Write(VISA resource name=w385, write buffer="*OPC", error in (no error)=w384) -> (VISA resource name out=w397:refnum<visa-resource-name>, error out=w396:errorcluster)  [unwired: 1 out]
    n138 = call <instrlib>:"ESR.vi"("error in (no error)"=w396, "VISA resource name"=w397) -> ("error out"=w391:errorcluster, "ESR"=w395:u8, "VISA resource name out"=w390:refnum<visa-resource-name>)  [unwired: 5 in, 2 out]
    n139 = And(x=w395, y=u8 1) -> (x .and. y?=w394:u8)
    n140 = Not Equal To 0?(x=w394) -> (x != 0?=w386:bool)
    "Complete?" <- w386
    n141 = call <instrlib>:"Print.vi"("Byte Count (1024)"=u32 256, "error in (no error)"=w391, "Input"=w399, "VISA resource name"=w390) -> ("error out"=w408:errorcluster, "Output"=w410:string, "VISA resource name out"=w405:refnum<visa-resource-name>)  [unwired: 3 in, 2 out]
    n142 = Scan From String(format string="%d %d", input string=w410, error in=w408) -> (error out=w404:errorcluster, output 1=w407:i32, output 2=w406:i32)  [unwired: 3 in, 2 out]
    n143 = Max & Min(x=w407, y=w406) -> (min(x,y)=w379:i32)  [unwired: 1 out]
    n144 = Decrement(x=w379) -> (x-1=w389:i32)
    n145 = Greater Or Equal?(x=w379, y=w378) -> (x >= y?=w403:bool)
    n146 = Equal?(x=w379, y=w378) -> (x = y?=w377:bool)
    n147 = case shown="False" w403 {
      tunnel: w401 -> [w417 w444]
      tunnel: w405 -> [w420 w443]
      tunnel: w404 -> [w421 w442]
      tunnel: w389 -> [w427 w441]
      tunnel: w378 -> [w434 w440]
      tunnel: u32 4096 ("Byte Count (1024)") -> [w433 w439]
      tunnel: [w423 w438] -> w381
      tunnel: [w416 w436] -> w382
      tunnel: [w415 w437] -> w398
      tunnel: w377 -> [_ w435]
      frame False {
        n148 = VISA Write(VISA resource name=w420, write buffer="i_ds.clearcache()\nv_ds.clearcache()" ("format string"), error in (no error)=w421) -> (VISA resource name out=w419:refnum<visa-resource-name>, error out=w418:errorcluster)  [unwired: 1 out]
        n149 = local read "Buffer size"() -> (w432:u32)
        n150 = call <instrlib>:"Print Buffer.vi"("VISA resource name"=w419, "Start Index (1)"=w434, "End Index (1)"=w432, "Buffer Name(s)"=w417, "error in (no error)"=w418, "Byte Count (1024)"=w433) -> ("VISA resource name out"=w430:refnum<visa-resource-name>, "Buffer Data"=w431:string, "error out"=w429:errorcluster)  [unwired: 5 in, 2 out]
        n151 = call <instrlib>:"Real 32 Converter.vi"("Data In"=w431) -> ("Data Array Out"=w425:sgl[])  [unwired: 10 in]
        n152 = call <instrlib>:"Print Buffer.vi"("VISA resource name"=w430, "Start Index (1)"=u32 1, "End Index (1)"=w427, "Buffer Name(s)"=w417, "error in (no error)"=w429) -> ("VISA resource name out"=w415:refnum<visa-resource-name>, "Buffer Data"=w426:string, "error out"=w416:errorcluster)  [unwired: 6 in, 2 out]
        n153 = call <instrlib>:"Real 32 Converter.vi"("Data In"=w426) -> ("Data Array Out"=w424:sgl[])  [unwired: 10 in]
        n154 = Build Array (concatenate)(w425, w424) -> (w423:sgl[])
      }
      frame True {
        n155 = case shown="True" w435 {
          tunnel: w444 -> [w454 _]
          tunnel: w443 -> [w453 w457]
          tunnel: w442 -> [w452 w456]
          tunnel: w441 -> [w451 _]
          tunnel: w440 -> [w450 _]
          tunnel: w439 -> [w449 _]
          tunnel: [w447 sgl[] [] ("Data Array Out")] -> w438
          tunnel: [w446 w457] -> w437
          tunnel: [w445 w456] -> w436
          frame False {
            n156 = call <instrlib>:"Print Buffer.vi"("VISA resource name"=w453, "Start Index (1)"=w450, "End Index (1)"=w451, "Buffer Name(s)"=w454, "error in (no error)"=w452, "Byte Count (1024)"=w449) -> ("VISA resource name out"=w446:refnum<visa-resource-name>, "Buffer Data"=w448:string, "error out"=w445:errorcluster)  [unwired: 5 in, 2 out]
            n157 = call <instrlib>:"Real 32 Converter.vi"("Data In"=w448) -> ("Data Array Out"=w447:sgl[])  [unwired: 10 in]
          }
          frame True {
          }
        }
      }
    }
    n158 = Empty Array?(array=w381) -> (empty?=w380:bool)
    n159 = case shown="False" w380 {
      tunnel: w383 -> [w413 _]
      tunnel: w381 -> [w412 _]
      frame False {
        n160 = Lossy Enqueue Element(queue=w413, element=w412) -> (overflow?=→"Overflow?":bool)  [unwired: 1 in, 3 out]
      }
      frame True {
      }
    }
    n161 = Or(x=w386, y="Stop") -> (x .or. y?=w387:bool)
  }
  n162 = Release Queue(queue=w29) -> (error out=w26:errorcluster)  [unwired: 2 in, 2 out]
  n163 = Decimate 1D Array(w15) -> (w18:sgl[], w17:sgl[], w16:sgl[])
  n164 = for {
    tunnel: w18 -> [w463] mode=indexing
    tunnel: w17 -> [w459] mode=indexing
    tunnel: w16 -> [w462] mode=indexing
    n165 = To Time Stamp(1:w459) -> (0:w464:timestamp)
    n166 = Build Array(w463) -> (w461:sgl[])
    n167 = Build Array(w462) -> (w460:sgl[])
    n168 = Bundle By Name("Y"=w461, "t0"=w464) -> (w466:waveform(sgl))  [unwired: 1 in]
    n169 = Bundle By Name("Y"=w460, "t0"=w464) -> (w465:waveform(sgl))  [unwired: 1 in]
    n170 = Merge Signals(w466, w465) -> (w458:dynamicdata)
    n171 = local write "Result Chart"(w458) -> ()
  }
  n172 = case shown="False" w53 {
    tunnel: w61 -> [w474 w476]
    tunnel: w60 -> [w473 w475]
    tunnel: [w468 w476] -> w59
    tunnel: [w467 w475] -> w58
    frame False {
      w469 = u16 1 items=["Channel A", "Channel B"] ("Channel (Channel A)")
      w470 = u16 0 items=["Channel A", "Channel B"] ("Channel (Channel A)")
      # "Abort Operation"
      n173 = call <instrlib>:"Abort SMU Op.vi"("error in"=w473, "Channel (Channel A)"=w470, "VISA resource name"=w474) -> ("error out"=w471:errorcluster, "VISA resource name out"=w472:refnum<visa-resource-name>)  [unwired: 5 in, 2 out]
      n174 = call <instrlib>:"Abort SMU Op.vi"("error in"=w471, "Channel (Channel A)"=w469, "VISA resource name"=w472) -> ("error out"=w467:errorcluster, "VISA resource name out"=w468:refnum<visa-resource-name>)  [unwired: 5 in, 2 out]
    }
    frame True {
      # "Operation Completed"
    }
  }
  n175 = local read "Auto Enable Output"() -> (w11:bool)
  n176 = case shown="False" w11 {
    tunnel: w59 -> [w478 w482]
    tunnel: w58 -> [w477 w481]
    tunnel: [w477 w480] -> w55
    tunnel: [w478 w479] -> w54
    frame False {
    }
    frame True {
      w487 = FALSE ("Output (Off)")
      n177 = local read "Drain Source Channel"() -> (w484:T1)
      n178 = local read "Pulse Channel"() -> (w483:T1)
      n179 = call <instrlib>:"Source Output Enable.vi"("Output (Off)"=w487, "error in (no error)"=w481, "Channel (Channel A)"=w484, "VISA resource name"=w482) -> ("error out"=w485:errorcluster, "VISA resource name out"=w486:refnum<visa-resource-name>)  [unwired: 4 in, 2 out]
      n180 = call <instrlib>:"Source Output Enable.vi"("Output (Off)"=w487, "error in (no error)"=w485, "Channel (Channel A)"=w483, "VISA resource name"=w486) -> ("error out"=w480:errorcluster, "VISA resource name out"=w479:refnum<visa-resource-name>)  [unwired: 4 in, 2 out]
    }
  }
  n181 = case shown="True" w53 {
    tunnel: w55 -> [w488 w507]
    tunnel: w54 -> [w489 w506]
    tunnel: [w488 w495] -> w52
    tunnel: [w489 w501] -> w51
    frame False {
      # "Operation Aborted, do nothing"
    }
    frame True {
      # "Plot and save Pulsed IV (single point)"
      n182 = local read "Pulse Number"() -> (w503:u32)
      n183 = call <instrlib>:"Print Buffer.vi"("VISA resource name"=w506, "End Index (1)"=w503, "Buffer Name(s)"="pulse_iv_table.v, pulse_iv_table.i" ("Buffer Name (buf)"), "error in (no error)"=w507, "Byte Count (1024)"=u32 4096) -> ("VISA resource name out"=w501:refnum<visa-resource-name>, "Buffer Data"=w502:string, "error out"=w496:errorcluster)  [unwired: 6 in, 2 out]
      n184 = call <instrlib>:"Real 32 Converter.vi"("Data In"=w502) -> ("Data Array Out"=w500:sgl[])  [unwired: 10 in]
      n185 = Decimate 1D Array(w500) -> (w499:sgl[], w498:sgl[])
      n186 = call "Convert to Dynamic Data2"("Array"=w498) -> ("Dynamic Data Type"=w493:dynamicdata)  [unwired: 3 in]
      n187 = call "Convert to Dynamic Data"("Array"=w499) -> ("Dynamic Data Type"=w494:dynamicdata)  [unwired: 3 in]
      n188 = Merge Signals(w494, w493) -> (w490:dynamicdata)
      n189 = call "Build XY Graph"("error in (no error)"=w496, "Y Input"=w493, "X Input"=w494) -> ("error out"=w495:errorcluster, "XY Graph"=→"Pulse IV":cluster{"X":dbl[], "Y":dbl[]}[])  [unwired: 7 in]
      n190 = call "Write To Measurement File2"("Signals"=w490, "Filename"="Pulsed IV Filename") -> ("Filename Out"=→"Pulsed IV Filename Out":path)  [unwired: 15 in, 2 out]
    }
  }
  n191 = call <instrlib>:"Close.vi"("error in (no error)"=w52, "VISA resource name"=w51) -> ("error out"=w28:errorcluster)  [unwired: 9 in]
  n192 = Merge Errors(w28, w26) -> (→"error out":errorcluster)
